vi "VIH - VI Doc Editor #2 - Get Nested GenObject Refnums.vi"(7 "Expand Tab Control (T)":bool=TRUE, 8 "error in":errorcluster, 9 "Skip Cluster if it's Array element (F)":bool, 11 "Gen Refnum":refnum<vi>) -> (0 "error out":errorcluster, 2 "Gen Refnums":refnum<vi>[](array[refnum]), 3 "dup Gen Refnum":refnum<vi>)   [LabVIEW 2014]
doc: "::: VI Helpeks :::\nCopyright (c) 2000-2026 Konstantin Shifershteyn. All rights reserved."
panel:
  # "VI Helpeks\nCopyright (c) 2012-2026 Konstantin Shifershteyn"
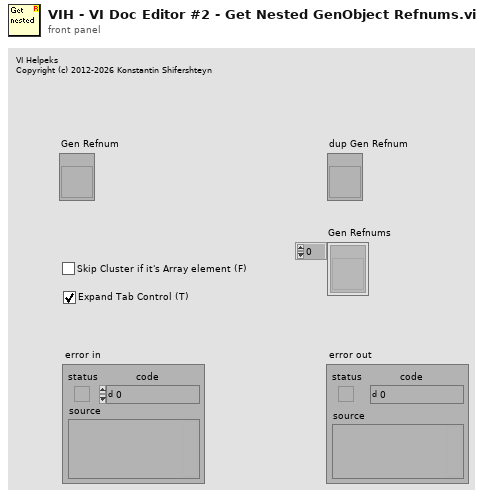
[diagram p1: front panel]
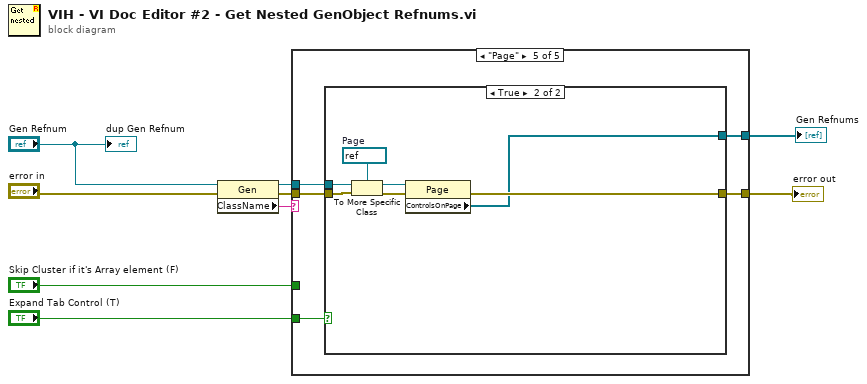
[diagram p0: block diagram]
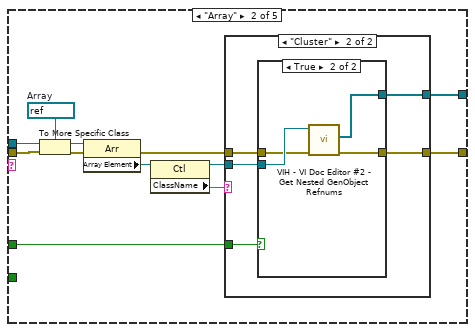
[diagram p3: hidden frame]
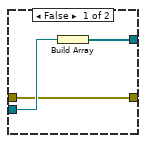
[diagram p5: hidden frame]
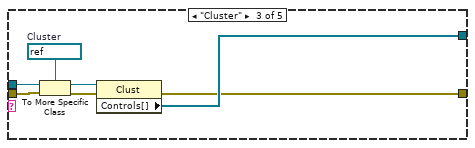
[diagram p6: hidden frame]
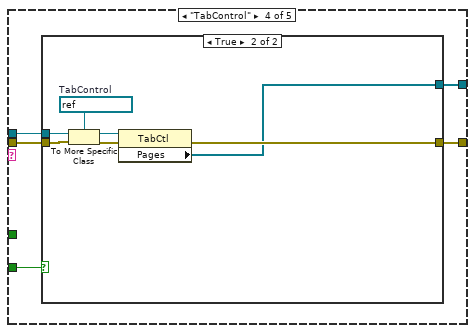
[diagram p7: hidden frame]
diagram:
  n1 = property class="Gen"(reference="Gen Refnum", error in="error in") -> (reference out=w3:refnum<vi>, error out=w2:errorcluster, "ClassName"=w1:string)
  n2 = case shown="\"Page\"" w1 {
    tunnel: w3 -> [_ w22 w42 w47 w60]
    tunnel: w2 -> [w10 w21 w41 w46 w59]
    tunnel: [_ w20 w40 w44 w57] -> w7
    tunnel: [w10 w12 w39 w45 w58] -> w6
    tunnel: "Skip Cluster if it's Array element (F)" -> [_ w11 _ _ _]
    tunnel: "Expand Tab Control (T)" -> [_ _ _ w43 w56]
    frame Default {
    }
    frame "Array" {
      w17 = refnum<vi> refnum  # Array
      n3 = To More Specific Class(target class=w17, reference=w22, error in=w21) -> (specific class reference=w18:refnum<vi>, error out=w19:errorcluster)
      n4 = property class="Arr"(reference=w18, error in=w19) -> (error out=w13:errorcluster, "Array Element"=w16:refnum<vi>)  [unwired: 1 out]
      n5 = property class="Ctl"(reference=w16) -> (reference out=w15:refnum<vi>, "ClassName"=w14:string)  [unwired: 1 in, 1 out]
      n6 = case shown="\"Cluster\"" w14 {
        tunnel: [_ w28] -> w20
        tunnel: w15 -> [_ w27]
        tunnel: w13 -> [w23 w26]
        tunnel: [w23 w25] -> w12
        tunnel: w11 -> [_ w24]
        frame Default {
        }
        frame "Cluster" {
          n7 = case shown="True" w24 {
            tunnel: [w31 w34] -> w28
            tunnel: w27 -> [w30 w35]
            tunnel: w26 -> [w29 w33]
            tunnel: [w29 w32] -> w25
            frame False {
              n8 = Build Array(w30) -> (w31:refnum<vi>[])
            }
            frame True {
              n9 = call "VIH - VI Doc Editor #2 - Get Nested GenObject Refnums.vi"("error in"=w33, "Gen Refnum"=w35) -> ("error out"=w32:errorcluster, "Gen Refnums"=w34:refnum<vi>[])  [unwired: 7 in, 1 out]
            }
          }
        }
      }
    }
    frame "Cluster" {
      w36 = refnum<vi> refnum  # Cluster
      n10 = To More Specific Class(target class=w36, reference=w42, error in=w41) -> (specific class reference=w37:refnum<vi>, error out=w38:errorcluster)
      n11 = property class="Clust"(reference=w37, error in=w38) -> (error out=w39:errorcluster, "Controls[]"=w40:refnum<vi>[])  [unwired: 1 out]
    }
    frame "TabControl" {
      n12 = case shown="True" w43 {
        tunnel: w47 -> [_ w52]
        tunnel: w46 -> [w48 w51]
        tunnel: [w48 w50] -> w45
        tunnel: [_ w49] -> w44
        frame False {
        }
        frame True {
          w53 = refnum<vi> refnum  # TabControl
          n13 = To More Specific Class(target class=w53, reference=w52, error in=w51) -> (specific class reference=w54:refnum<vi>, error out=w55:errorcluster)
          n14 = property class="TabCtl"(reference=w54, error in=w55) -> (error out=w50:errorcluster, "Pages"=w49:refnum<vi>[])  [unwired: 1 out]
        }
      }
    }
    frame "Page" {
      n15 = case shown="True" w56 {
        tunnel: w60 -> [_ w65]
        tunnel: w59 -> [w61 w64]
        tunnel: [w61 w63] -> w58
        tunnel: [_ w62] -> w57
        frame False {
        }
        frame True {
          w66 = refnum<vi> refnum  # Page
          n16 = To More Specific Class(target class=w66, reference=w65, error in=w64) -> (specific class reference=w67:refnum<vi>, error out=w68:errorcluster)
          n17 = property class="Page"(reference=w67, error in=w68) -> (error out=w63:errorcluster, "ControlsOnPage"=w62:refnum<vi>[])  [unwired: 1 out]
        }
      }
    }
  }
  "error out" <- w6
  "Gen Refnums" <- w7
  "dup Gen Refnum" <- "Gen Refnum"
